vi "VI Script - Set Message Queue.vi"() -> ()   [LabVIEW 2026]
doc: "Create All Message Queues.viã§ä½æããã­ã¥ã¼éåãã¯ã©ã¹ã¿ã«è¨­å®ãã¾ããZ²z"
uses:
  support/Message Queue/All Message Queues.ctl
  support/Message Queue/Message Cluster.ctl
  support/Message Queue/Create All Message Queues.vi
  support/Message Queue/Message Queue.lvlib
panel:
  out "error out":errorcluster
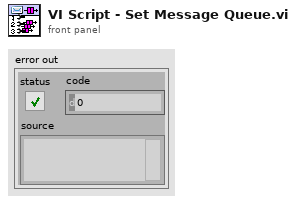
[diagram p1: front panel]
types:
  T1 = typedef "Message Queue.lvlib/All Message Queues.ctl" = cluster{"UI":refnum<queue>}
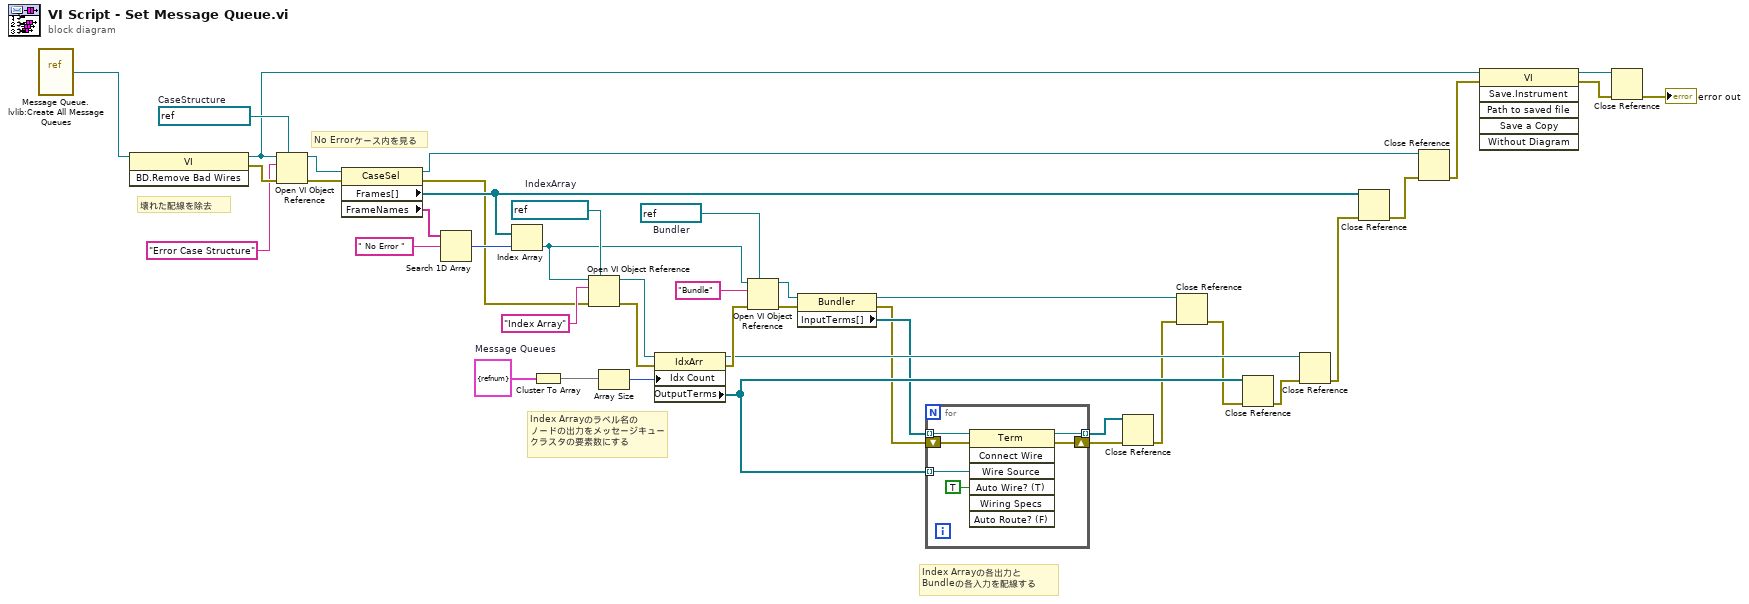
[diagram p0: block diagram]
diagram:
  w28 = refnum<vi> refnum  # IndexArray
  w19 = refnum<vi> refnum  # Bundler
  w37 = refnum<vi> refnum  # CaseStructure
  w40 = T1 {"UI"=refnum}  # Message Queues
  # "Index Arrayの各出力と\nBundleの各入力を配線する"
  # "Index Arrayのラベル名の\nノードの出力をメッセージキュー\nクラスタの要素数にする"
  # "No Errorケース内を見る"
  # "壊れた配線を除去"
  n1 = vi-ref "Message Queue.lvlib:Create All Message Queues.vi"() -> (w5:refnum<vi>)
  n2 = invoke class="VI" method="BD.Remove Bad Wires"(reference=w5) -> (reference out=w4:refnum<vi>, error out=w39:errorcluster)  [unwired: 2 in, 1 out]
  n3 = Open VI Object Reference(7:w37, 8:w39, 10:"Error Case Structure" ("name/order"), 11:w4) -> (0:w35:errorcluster, 3:w36:refnum<vi>)
  n4 = property class="CaseSel"(reference=w36, error in=w35) -> (reference out=w34:refnum<vi>, error out=w26:errorcluster, "Frames[]"=w30:refnum<vi>[], "FrameNames"=w32:string[])
  n5 = Search 1D Array(1D array=w32, element=" No Error ") -> (index of element=w31:i32)  [unwired: 1 in]
  n6 = Index Array(array=w30, index=w31) -> (element=w20:refnum<vi>)
  n7 = Cluster To Array(cluster=w40) -> (array=w41:refnum<queue>[])
  n8 = Open VI Object Reference(7:w28, 8:w26, 10:"Index Array", 11:w20) -> (0:w24:errorcluster, 3:w25:refnum<vi>)
  n9 = Array Size(array=w41) -> (size(s)=w23:i32)
  n10 = property class="IdxArr"(reference=w25, error in=w24, "Idx Count"=w23) -> (reference out=w16:refnum<vi>, error out=w21:errorcluster, "OutputTerms"=w15:refnum<vi>[])
  n11 = Open VI Object Reference(7:w19, 8:w21, 10:"Bundle" ("name/order"), 11:w20) -> (0:w7:errorcluster, 3:w13:refnum<vi>)
  n12 = property class="Bundler"(reference=w13, error in=w7) -> (reference out=w8:refnum<vi>, error out=w6:errorcluster, "InputTerms[]"=w12:refnum<vi>[])
  n13 = for {
    tunnel: w15 -> [w46] mode=indexing
    shift-right: [w47] -> w17
    shift-left: w6 -> [w45]
    tunnel: w12 -> [w44] mode=indexing
    tunnel: [w43] -> w11 mode=indexing
    n14 = invoke class="Term" method="Connect Wire"(reference=w44, error in=w45, "Wire Source"=w46, "Auto Wire? (T)"=TRUE) -> (reference out=w43:refnum<vi>, error out=w47:errorcluster)  [unwired: 3 in, 5 out]
  }
  n15 = Close Reference(reference=w11, error in (no error)=w17) -> (error out=w10:errorcluster)
  n16 = Close Reference(reference=w8, error in (no error)=w10) -> (error out=w9:errorcluster)
  n17 = Close Reference(reference=w15, error in (no error)=w9) -> (error out=w14:errorcluster)
  n18 = Close Reference(reference=w16, error in (no error)=w14) -> (error out=w22:errorcluster)
  n19 = Close Reference(reference=w30, error in (no error)=w22) -> (error out=w29:errorcluster)
  n20 = Close Reference(reference=w34, error in (no error)=w29) -> (error out=w2:errorcluster)
  n21 = invoke class="VI" method="Save.Instrument"(reference=w4, error in=w2) -> (reference out=w3:refnum<vi>, error out=w1:errorcluster)  [unwired: 4 in, 4 out]
  n22 = Close Reference(reference=w3, error in (no error)=w1) -> (error out=→"error out":errorcluster)
